vi "FluidtekPrensaCONidentLEDI_v15.vi"() -> ()   [LabVIEW 2026]
uses:
  <vilib>/DAQmx/read.llb/DAQmx Read (Digital 1D Bool NChan 1Samp 1Line).vi
  <vilib>/DAQmx/write.llb/DAQmx Write (Digital 1D Bool NChan 1Samp 1Line).vi
  <vilib>/DAQmx/read.llb/DAQmx Read (Analog 1D Wfm NChan NSamp).vi
  <vilib>/Analysis/baseanly.llb/Mean (DBL).vi
  <vilib>/DAQmx/write.llb/DAQmx Write (Analog DBL 1Chan 1Samp).vi
  <extravilib>/ChannelInstances/Tag-bool/Read With Abort.vi
  <extravilib>/ChannelInstances/Tag-c(dbl,dbl,dbl,dbl,dbl,dbl)/Read With Abort.vi
  <extravilib>/ChannelInstances/Tag-c(dbl,dbl,dbl,dbl,dbl,dbl,dbl,bool,u16)/Write With Abort.vi
  <extravilib>/ChannelInstances/Tag-bool/Write With Abort.vi
  <extravilib>/ChannelInstances/Tag-c(dbl,dbl,dbl,dbl,dbl,dbl,dbl,bool,u16)/Read With Abort.vi
  <extravilib>/ChannelInstances/Tag-c(dbl,dbl,dbl,dbl,dbl,dbl)/Write With Abort.vi
  GlobalesPrensa.vi
  <vilib>/Utility/file.llb/Write Delimited Spreadsheet (DBL).vi
  <vilib>/DAQmx/create/channels.llb/DAQmx Create Channel (AO-Voltage-Basic).vi
  <vilib>/DAQmx/create/channels.llb/DAQmx Create Channel (AI-Voltage-Basic).vi
  <vilib>/DAQmx/configure/timing.llb/DAQmx Timing (Sample Clock).vi
  <vilib>/DAQmx/create/channels.llb/DAQmx Create Channel (DO-Digital Output).vi
  <vilib>/DAQmx/create/channels.llb/DAQmx Create Channel (DI-Digital Input).vi
  <extravilib>/ChannelInstances/Tag-bool/Instantiate.vi
  <extravilib>/ChannelInstances/Tag-bool/Endpoint.vi
  <vilib>/DAQmx/miscellaneous.llb/DAQmx Fill In Error Info.vi
  <extravilib>/ChannelInstances/Tag-c(dbl,dbl,dbl,dbl,dbl,dbl,dbl,bool,u16)/Instantiate.vi
  <extravilib>/ChannelInstances/Tag-c(dbl,dbl,dbl,dbl,dbl,dbl)/Instantiate.vi
  <extravilib>/ChannelInstances/Tag-bool/EndpointRead.vi
  <extravilib>/ChannelInstances/Tag-c(dbl,dbl,dbl,dbl,dbl,dbl)/EndpointRead.vi
  <extravilib>/ChannelInstances/Tag-c(dbl,dbl,dbl,dbl,dbl,dbl,dbl,bool,u16)/Endpoint.vi
  <extravilib>/ChannelInstances/Tag-c(dbl,dbl,dbl,dbl,dbl,dbl,dbl,bool,u16)/EndpointRead.vi
  <extravilib>/ChannelInstances/Tag-c(dbl,dbl,dbl,dbl,dbl,dbl)/Endpoint.vi
  <vilib>/Analysis/NI_AALBase.lvlib
  <extravilib>/ChannelInstances/Tag-bool.lvlib
  <extravilib>/ChannelInstances/Tag-c(dbl,dbl,dbl,dbl,dbl,dbl).lvlib
  <vilib>/ptbypt/NI_PtbyPt.lvlib
  <extravilib>/ChannelInstances/Tag-c(dbl,dbl,dbl,dbl,dbl,dbl,dbl,bool,u16).lvlib
panel:
  out "Archivo":path
  out "Lg log":dbl[](array[numeric])
  in  "PARO DE EMERGENCIA":bool
  out "time/iteration (ms)":u32=210
  in  "Tab Control 3":enum32{"ENSAYO", "REGISTRO"}(tab)
  in  "Tipo ensayos":u16(ring)=1 items=["Flexotraccion en losas", "Tenacidad Vigas"]
  in  "Rampa (mm/min)":dbl=0.1 min=0.0 max=25.0 format="%.3f"
  in  "Rampa (kN/min)":dbl=0.1 min=0.0 max=20.0 format="%.2f"
  in  "Limite fuerza (kN)":dbl=3.0 min=0.0 max=150.0 format="%.2f"
  in  "Limite posicion (mm)":dbl=145.0 min=0.0 max=150.0 format="%.2f"
  in  "Tiempo carga (s)":dbl=3.0 min=0.0 max=300.0 format="%.2g"
  out "Tiempo (s)":dbl format="%.2f"
  in  "Iniciar ensayo":bool
  out "Velocidad norma (mm/min)  2":string="0.05 - 0.1"
  in  "Tenacidad en vigas":u16(ring) items=["ASTM 1609 con100x100x350", "ASTM 1609 con150x150x500", "EFNARC 1996", "VIGAS 14651", "ENS. BARCELONA"]
  in  "Aplicar velocidad de norma":bool
  out "Estado del ensayo":dbl(ring) items=["REPOSO", "CARGA (rampa)", "MANTENIENDO CARGA", "DESCARGA", "RETORNO / FIN", "FALLA - ENSAYO DETENIDO", ""]
  in  "Flexotracción en losas":u16(ring)=3 items=["EFNARC 1996", "EFNARC 1999", "EFNARC 14488-5", "ASTM 1550"]
  out "Velocidad norma (mm/min)":dbl=4.0
  in  "IPAddress QuantumX":string="172.31.236.115"
  out "LicenseIsValid":bool
  in  "Registrar":bool
  in  "ID manual (0=auto)":i32
  in  "Tipo":string
  in  "INFLE":dbl
  in  "Detener registro":bool
  in  "Tab Control 2":T1(tab)
  out "Presión B (bar)":dbl=31.47939829954219 format="%.2f"
  out "Presión A (bar)":dbl=47.7049180327869 format="%.2f"
  out "Vertical Progress Bar":dbl(slide)=3.0
  in  "Tab Control":enum32{"Desplazamiento", "Fuerza"}(tab)
  in  "PID fuerza":T2={"proportional gain (Kc)"=1.0, "integral time (Ti, min)"=0.03, "derivative time (Td, min)"=0.0} {"derivative time (Td, min)" format="%.3f"; "integral time (Ti, min)" format="%.3f"; "proportional gain (Kc)" format="%.3f"}
  out "control signals":dynamicdata(graph)=[{"t0"=timestamp(3594752785.1434503 s since 1904-01-01), "dt"=1.0, "Y"=[3.0]}, {"t0"=timestamp(3594752785.1434503 s since 1904-01-01), "dt"=1.0, "Y"=[3.0680651042487943]}]
  in  "Posicion deseada (mm)":dbl(slide)=3.0 min=2.0 max=150.0 scale format="%#_2f"
  in  "Fuerza deseada (kN)":dbl=0.5 min=0.0 max=150.0 format="%.2f"
  out "Fuerza actual (KN)":dbl format="%.2f"
  out "Posicion actual (mm)":dbl format="%.2f"
  in  "Tipo control":u16(ring) items=["Desplazamiento", "Fuerza"]
  out "fuerza desplazamiento":cluster{dbl[], dbl[]}(graph)
  out "Rigidez estimada (kN/mm)":dbl
  out "Carga maxima (kN)":dbl
  out "Progreso mantenimiento":dbl(slide) scale=0.0..100.0
  out "Tiempo restante carga (s)":dbl
  out "Falla":bool
  out "Causa de la falla":dbl(ring) items=["Sin falla", "CAIDA DE CARGA (rotura)", "SOBRECARGA", "LIMITE DE POSICION", "PARO DE EMERGENCIA", "LIMITE DEL SISTEMA (160 kN)", "SIN LECTURA DE FUERZA (QuantumX)", "LIMITE POR PRESIONES (160 kN)"]
  out "Proteccion de fuerza activa":bool
  in  "Vel. aproximacion (mm/min)":dbl=50.0 min=0.1 max=50.0
  in  "Fmax fuera de ensayo (kN)":dbl=1.0 min=0.2 max=50.0
  out "UPH energizada":bool=TRUE
  out "Nivel tanque":bool
  out "Estado de  filtro":bool=TRUE
  out "Sobrecorriente":bool
  in  "Stop":bool
  out "Estado de motor":bool
  in  "Apagar":bool
  in  "Encender":bool
  in  "Sin proteccion de carga":bool
  in  "Confirmar parametros":bool=TRUE
  out "Consigna posicion interna (mm)":dbl
  out "Parametros avanzados":dbl(ring) items=["POR DEFECTO (bloqueados)", "PERSONALIZADOS (activos)"]
  in  "Codigo acceso":dbl
  in  "Sobrecarga falla (x limite)":dbl=1.2
  in  "Caida para falla (0-1)":dbl=0.3
  in  "Rigidez inicial (kN/mm)":dbl=1.0
  in  "Kf lazo fuerza (1/s)":dbl=0.5
  in  "Kx lazo posicion (V/mm)":dbl=30.0
  in  "Ti lazo posicion (s)":dbl=1.5
  # "PB"
  # "PA"
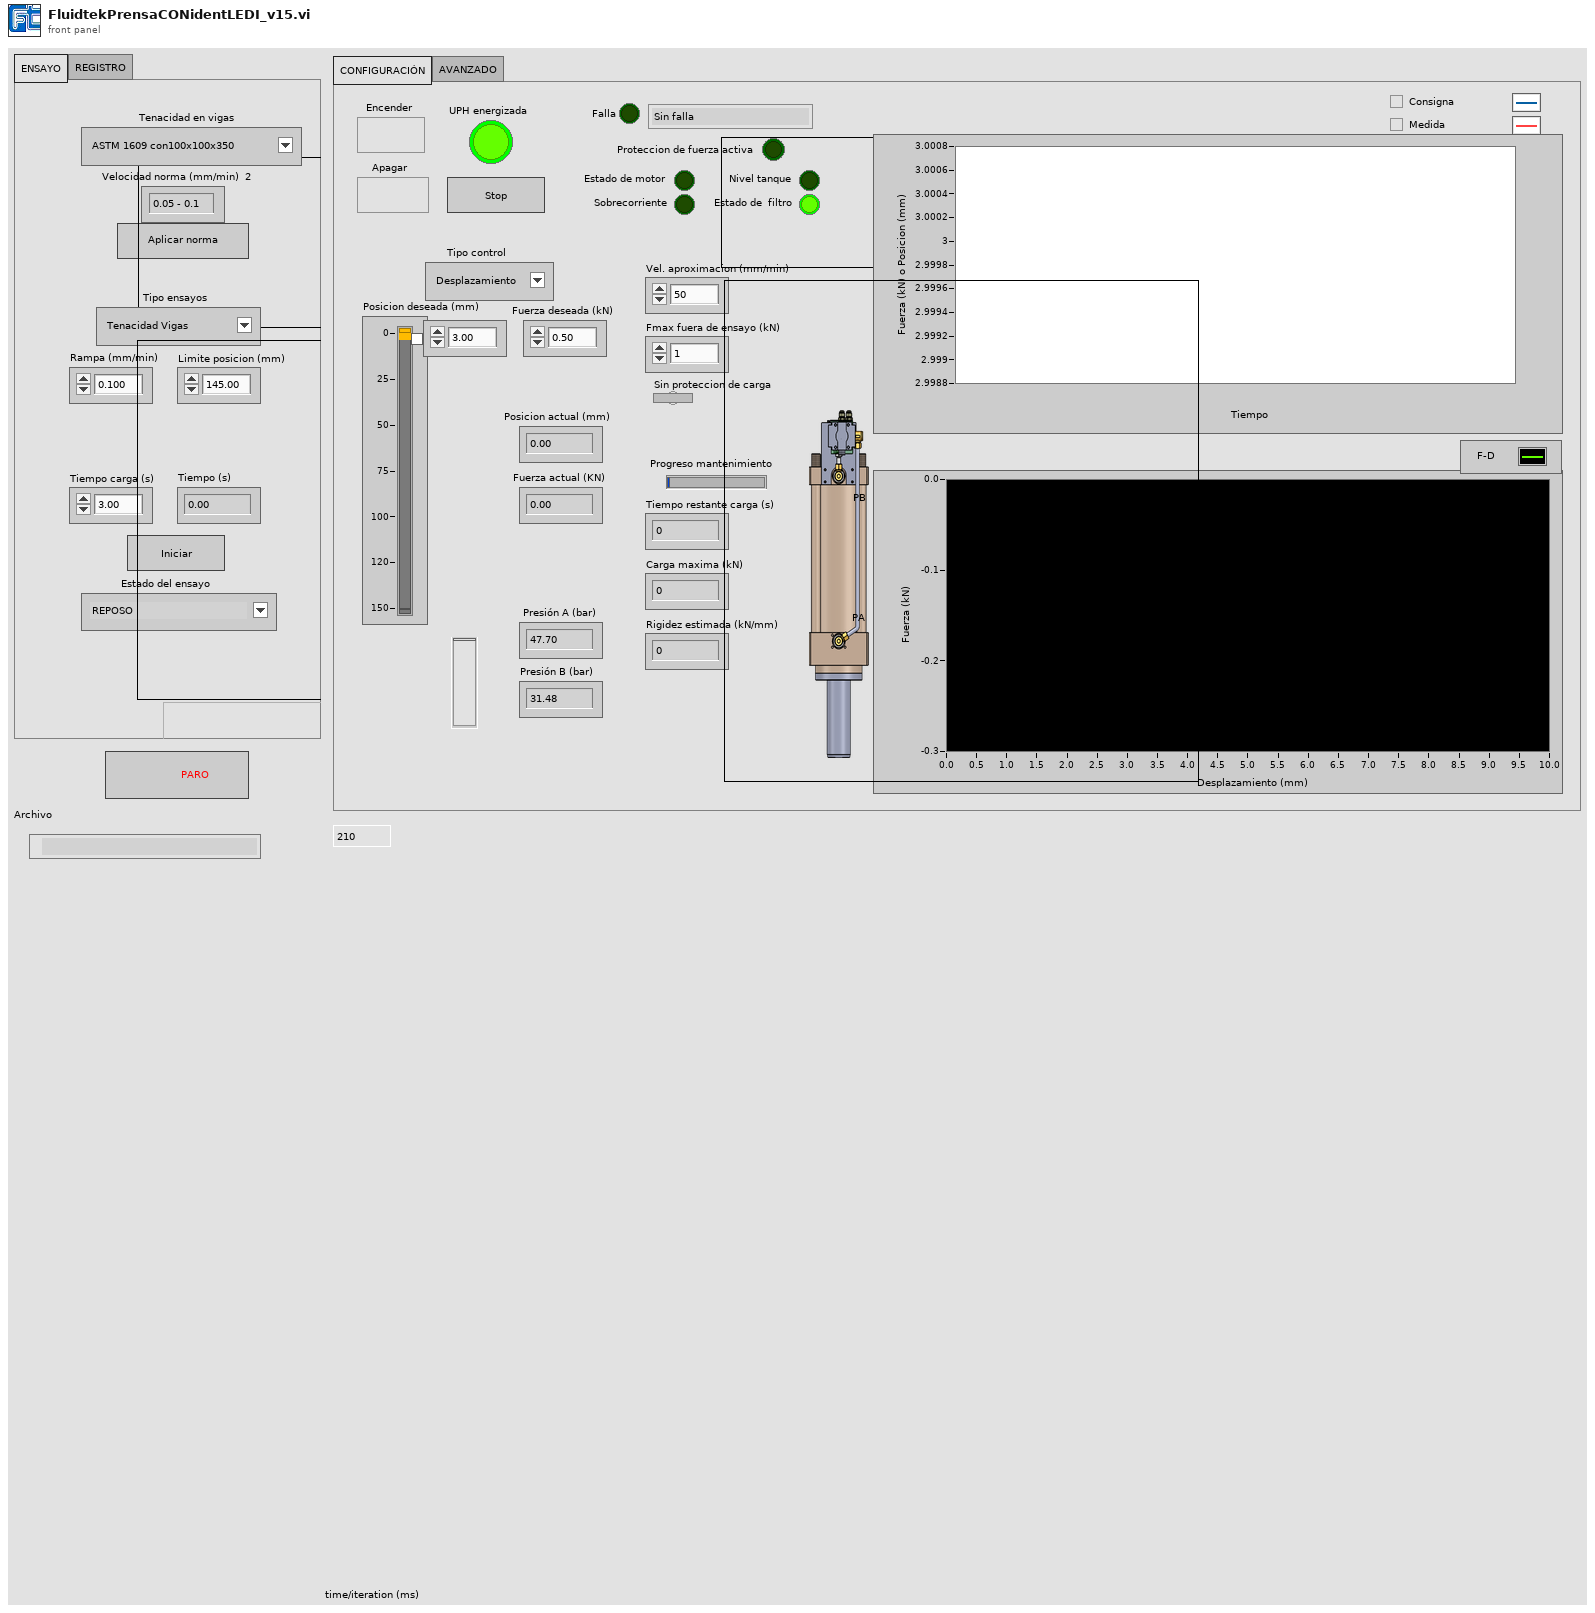
[diagram p1: front panel]
types:
  T1 = enum32{"CONFIGURACIÓN", "AVANZADO", "identificación (no modificar)"}
  T2 = cluster{"proportional gain (Kc)":dbl, "integral time (Ti, min)":dbl, "derivative time (Td, min)":dbl}
  T3 = typedef "Tag-bool.lvlib/))Channel.ctl" = refnum<queue>
  T4 = cluster{"Devices":refnum<k24>[], "Signals":refnum<k24>[]}
  T5 = cluster{"Rampa (mm/min)":dbl, "Rampa (kN/min)":dbl, "Limite posicion (mm)":dbl, "Limite fuerza (kN)":dbl, "Posicion deseada (mm)":dbl, "Fuerza deseada (kN)":dbl, "Tiempo carga (s)":dbl, "Iniciar ensayo":bool, "Tipo control":u16}
  T6 = cluster{"Numeric":dbl, "mean":dbl, "mean":dbl, "mean":dbl, "mean":dbl, "sp":dbl}
  T7 = typedef "Tag-c(dbl,dbl,dbl,dbl,dbl,dbl).lvlib/))Channel.ctl" = refnum<queue>
  T8 = enum8{"Enabled", "Disabled", "Disabled and Grayed Out"}
  T9 = cluster{"Numeric":dbl, dbl, dbl, dbl, dbl, "Limite fuerza (kN)":dbl}
  T10 = typedef "Tag-c(dbl,dbl,dbl,dbl,dbl,dbl,dbl,bool,u16).lvlib/))Channel.ctl" = refnum<queue>
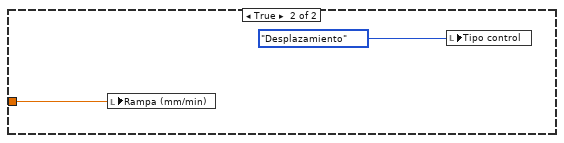
[diagram p5: hidden frame]
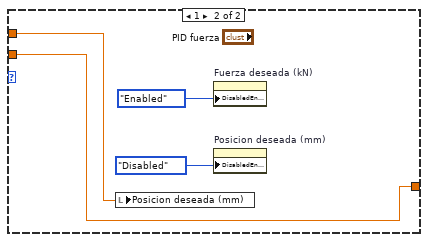
[diagram p6: hidden frame]
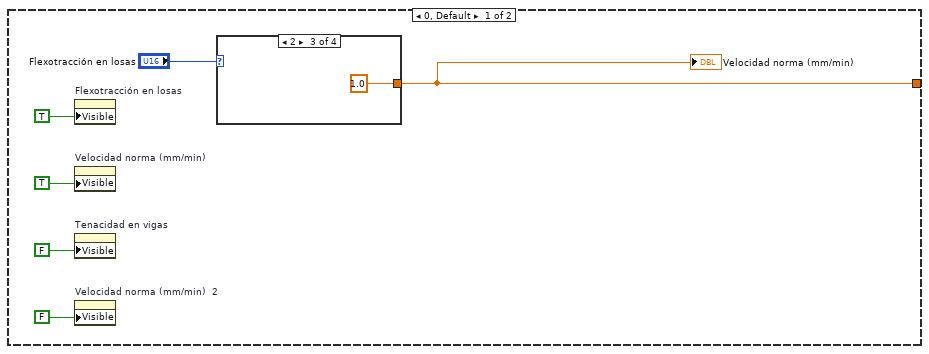
[diagram p7: hidden frame]
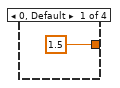
[diagram p8: hidden frame]
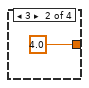
[diagram p9: hidden frame]
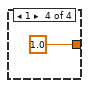
[diagram p10: hidden frame]
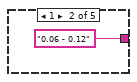
[diagram p11: hidden frame]
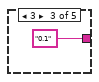
[diagram p12: hidden frame]
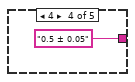
[diagram p13: hidden frame]
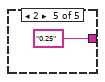
[diagram p14: hidden frame]
diagram:
  w76 = 0 items=["one channel for each line", "one channel for all lines"] ("line grouping")
  w83 = 0 items=["one channel for each line", "one channel for all lines"] ("line grouping")
  w95 = 10348 items=["Volts"=10348, "From Custom Scale"=10065] ("units")
  w98 = -1 items=["Default"=-1, "RSE"=10083, "NRSE"=10078, "Differential"=10106, "Pseudodifferential"=12529] ("input terminal configuration")
  w106 = 10348 items=["Volts"=10348, "From Custom Scale"=10065] ("units")
  w104 = 10106 items=["Default"=-1, "RSE"=10083, "NRSE"=10078, "Differential"=10106, "Pseudodifferential"=12529] ("input terminal configuration")
  w100 = 10123 items=["Finite Samples"=10178, "Continuous Samples"=10123, "Hardware Timed Single Point"=12522] ("sample mode")
  # "Convert device reference to array of device references\n(since ConnectDevice.vi expects an array of devices)..."
  # "Disconnect devices"
  # "Set samplerate and filter frequency for all selected signals."
  # "Initialize HBM Common API for LabVIEW"
  # "End API usage"
  # "Stop DAQ"
  # "Run data acquisition for 10 sec. DAQ-loop: Update signals and do anything with the  measurement values.\n(Here: show first signal in diagram)"
  # "Start DAQ"
  # "Prepare DAQ"
  # "v14: senales [0,1,2,3] -> lazo lee 1,2,3 = W100 (conector 2), Tempsonic (conector 3), Celda via Krenel (conector 4). Filtro 20 Hz, 50 Hz"
  # "Get all signals of the devices"
  # "Connect devices"
  # "Use certain QuantumX device"
  # "Assign the signals...."
  # "Vel. aprox. (mm/min)"
  # "LAZO E/S DIGITAL: encendido/apagado de la unidad hidraulica (contactores), lectura de alarmas (motor, sobrecorriente, nivel, filtro)."
  # "LAZO HMI: lee el panel, habilita/oculta controles segun modo y estado, envia consignas al lazo de control por canal (Tag)."
  # "LAZO DE CONTROL: lectura DAQ (fuerza, desplazamiento, presiones) -> Formula Node 'CONTROLADOR' (maquina de estados + cascada fuerza/posicion + fallas) -> salida servovalvula (AO). Parametros avanzados protegidos con codigo."
  n1 = while {
    tunnel: [w111] -> w3
    tunnel: [w111] -> w2
    tunnel: [w111] -> w1
    i -> [w116]
    stop <- w114 continue-if-true
    n2 = call <vilib>:"DAQmx Reserve Network Device.vi"("device in"=tag "cDAQ9184-1ADC24C", "override reservation?"=TRUE, "error in"=errorcluster {"status"=FALSE, "code"=0, "source"=""}) -> ("error out"=w111:errorcluster)  [unwired: 11 in, 1 out]
    n3 = Unbundle By Name(w111) -> ("status"=w113:bool)
    n4 = Less?(x=w116, y=30) -> (x < y?=w115:bool)
    n5 = And(x=w113, y=w115) -> (x .and. y?=w114:bool)
    n6 = Wait (ms)(milliseconds to wait=u32 2000) -> ()  [unwired: 1 out]
  }
  n7 = call-poly <vilib>:"DAQmx Create Virtual Channel.vi"("lines"=tag "PrensaLEDI_DO/port0/line0:7", "line grouping"=w76, "error in"=w2) -> ("task out"=w77:refnum<k21>, "error out"=w78:errorcluster)  [unwired: 11 in]
  n8 = call-poly <vilib>:"DAQmx Create Virtual Channel.vi"("lines"=tag "PrensaLEDI_DI/port0/line0:7", "line grouping"=w83, "error in"=w3) -> ("task out"=w80:refnum<k21>, "error out"=w81:errorcluster)  [unwired: 11 in]
  n9 = call <vilib>:"DAQmx Start Task.vi"("task/channels in"=w77, "error in"=w78) -> ("task out"=w71:refnum<k21>, "error out"=w70:errorcluster)  [unwired: 12 in]
  n10 = call <vilib>:"DAQmx Start Task.vi"("task/channels in"=w80, "error in"=w81) -> ("task out"=w73:refnum<k21>, "error out"=w72:errorcluster)  [unwired: 12 in]
  n11 = while {
    tunnel: w73 -> [w132]
    tunnel: w72 -> [w131]
    tunnel: [w130] -> w56
    tunnel: [w129] -> w54
    tunnel: w71 -> [w128]
    tunnel: [w127] -> w60
    tunnel: w70 -> [w126]
    tunnel: [w125] -> w58
    tunnel: [w124] -> w6
    stop <- "Stop" stop-if-true
    # "6"
    # "APAGADO Y ENCENDIDO TIPO PULSO"
    # "transmisor de presion"
    # "salida contactor2"
    # "salida al contactor"
    # "pulsador\nemergencia"
    # "GM2"
    n12 = call-poly <vilib>:"DAQmx Read.vi"("task/channels in"=w132, "error in"=w131) -> ("task out"=w130:refnum<k21>, "data"=w147:bool[], "error out"=w129:errorcluster)  [unwired: 11 in]
    n13 = Index Array(array=w147, index=7) -> ()  [unwired: 1 out]
    n14 = global write "GlobalesPrensa.vi" "Salir"("Stop") -> ()
    n15 = Index Array(array=w147, index=5) -> (element=w156:bool)
    "Sobrecorriente" <- w156
    n16 = Index Array(array=w147, index=0) -> (element=w146:bool)
    n17 = Index Array(array=w147, index=2) -> (element=w148:bool)
    n18 = Not(x="Stop") -> (.not. x?=w145:bool)
    n19 = Not(x=w148) -> (.not. x?=→"Estado de  filtro":bool)
    n20 = Not(x=w156) -> (.not. x?=→"UPH energizada":bool)
    n21 = And(x=w146, y=w145) -> (x .and. y?=w152:bool)
    n22 = Index Array(array=w147, index=1) -> (element=→"Nivel tanque":bool)
    n23 = local read "PARO DE EMERGENCIA"() -> (w121:bool)
    n24 = Not(x=w152) -> (.not. x?=w153:bool)
    n25 = Not(x=w152) -> (.not. x?=w154:bool)
    n26 = Or(x="Apagar", y=w153) -> (x .or. y?=w122:bool)
    n27 = Or(x=w122, y=w121) -> (x .or. y?=w123:bool)
    n28 = while {
      shift-right: [w160] -> w157
      shift-left: _ -> [w162]
      tunnel: "Encender" -> [w161]
      tunnel: w123 -> [w159]
      stop <- FALSE continue-if-true
      n29 = Exclusive Or(1:w159, 2:w161) -> (0:w163:bool)
      n30 = Select(t=w161, s=w163, f=w162) -> (s? t:f=w160:bool)
    }
    "Estado de motor" <- w157
    n31 = Wait (ms)(milliseconds to wait=u32 500) -> ()  [unwired: 1 out]
    n32 = Replace Array Subset(array=bool[] [FALSE, FALSE, FALSE, FALSE, FALSE, FALSE, FALSE, FALSE], new element #1=w157, index #1=0 ("index"), new element #2=w154, index #2=2 ("index"), new element #3=TRUE ("new element/subarray"), index #3=5 ("index")) -> (w155:bool[])
    n33 = call-poly <vilib>:"DAQmx Write.vi"("task/channels in"=w128, "data"=w155, "error in"=w126) -> ("task out"=w127:refnum<k21>, "error out"=w125:errorcluster)  [unwired: 10 in, 1 out]
    n34 = call <extravilib>:"Write.vi"("element"="Stop") -> ("channel"=w124:T3)  [unwired: 1 out]
  }
  n35 = call-poly <vilib>:"DAQmx Create Virtual Channel.vi"("maximum value"=10.0, "minimum value"=0.0, "input terminal configuration"=w104, "physical channels"=tag "PrensaLEDI_AI/ai0:3", "units"=w106, "error in"=w1) -> ("task out"=w107:refnum<k21>, "error out"=w108:errorcluster)  [unwired: 8 in]
  n36 = call-poly <vilib>:"DAQmx Create Virtual Channel.vi"("maximum value"=10.0, "minimum value"=-10.0, "output terminal configuration"=w98, "physical channels"=tag "PrensaLEDI_AO/ao0", "units"=w95, "error in"=w1) -> ("task out"=w99:refnum<k21>, "error out"=w97:errorcluster)  [unwired: 8 in]
  n37 = call-poly <vilib>:"DAQmx Timing.vi"("task/channels in"=w107, "sample mode"=w100, "samples per channel"=500000, "rate"=200000.0, "error in"=w108) -> ("task out"=w68:refnum<k21>, "error out"=w67:errorcluster)  [unwired: 9 in]
  n38 = call <vilib>:"DAQmx Start Task.vi"("task/channels in"=w68, "error in"=w67) -> ("task out"=w66:refnum<k21>, "error out"=w65:errorcluster)  [unwired: 12 in]
  n39 = call <vilib>:"DAQmx Start Task.vi"("task/channels in"=w99, "error in"=w97) -> ("task out"=w88:refnum<k21>, "error out"=w87:errorcluster)  [unwired: 12 in]
  n40 = feedback-in #1(w6) -> ()
  n41 = feedback #1() -> ()  [unwired: 2 in]
  n42 = call <vilib>:"DAQmx Stop Task.vi"("task/channels in"=w60, "error in"=w58) -> ("task out"=w59:refnum<k21>, "error out"=w57:errorcluster)  [unwired: 12 in]
  n43 = call <vilib>:"DAQmx Stop Task.vi"("task/channels in"=w56, "error in"=w54) -> ("task out"=w55:refnum<k21>, "error out"=w53:errorcluster)  [unwired: 12 in]
  n44 = call <vilib>:"DAQmx Clear Task.vi"("task in"=w59, "error in"=w57) -> ("error out"=w75:errorcluster)  [unwired: 13 in]
  n45 = call <vilib>:"DAQmx Clear Task.vi"("task in"=w55, "error in"=w53) -> ("error out"=w74:errorcluster)  [unwired: 13 in]
  n46 = call <vilib>:"Simple Error Handler.vi"("error in (no error)"=w75) -> ()  [unwired: 4 in, 5 out]
  n47 = call <vilib>:"Simple Error Handler.vi"("error in (no error)"=w74) -> ()  [unwired: 4 in, 5 out]
  n48 = call <userlib>:"Init.vi"() -> ("LicenseIsValid"=→"LicenseIsValid":bool, "Error out"=w13:errorcluster)  [unwired: 8 in, 1 out]
  n49 = call <userlib>:"QuantumX_Device.vi"("Error in"=w13, "IPAddress"="IPAddress QuantumX") -> ("Error out"=w14:errorcluster, "Device"=w11:refnum<k24>)  [unwired: 6 in]
  n50 = Build Array(w11) -> (w10:refnum<k24>[])
  n51 = call <userlib>:"ConnectDevice.vi"("Error in"=w14, "Devices"=w10) -> ("Error out"=w36:errorcluster, "Devices"=w35:refnum<k24>[])  [unwired: 7 in, 1 out]
  n52 = call <userlib>:"GetSignals.vi"("Error in"=w36, "Devices"=w35) -> ("Error out"=w30:errorcluster, "DevicesAndSignals"=w31:T4)  [unwired: 8 in]
  n53 = Unbundle By Name(w31) -> ("Devices"=w24:refnum<k24>[], "Signals"=w28:refnum<k24>[])
  n54 = Index Array(array=w28, index #1=0 ("Index"), index #2=1 ("Index"), index #3=2 ("Index"), index #4=3 ("Index")) -> (element #1=w27:refnum<k24>, element #2=w26:refnum<k24>, element #3=w19:refnum<k24>, element #4=w18:refnum<k24>)
  n55 = Build Array(w27, w26, w19, w18) -> (w25:refnum<k24>[])
  n56 = Bundle(cluster=w31, "Devices"=w24, "Signals"=w25) -> (w32:T4)
  n57 = Unbundle By Name(w32) -> ("Signals"=w48:refnum<k24>[])
  n58 = case shown="No Error" w30 {
    tunnel: w30 -> [w169 w175]
    tunnel: w48 -> [w168 _]
    tunnel: [w167 w175] -> w47
    frame No Error {
      # "Filter frequency:"
      # "Samplerate:"
      n59 = for {
        tunnel: w169 -> [w174]
        tunnel: 50.0 ("SampleRate") -> [w173]
        tunnel: 20.0 ("FilterFrequency") -> [w172]
        tunnel: w168 -> [w171] mode=indexing
        tunnel: [w170] -> w167
        stop <- w170 stop-if-true
        n60 = call <userlib>:"ConfigSignal.vi"("Error in"=w174, "SampleRate"=w173, "FilterFrequency"=w172, "Signal"=w171) -> ("Error out"=w170:errorcluster)  [unwired: 7 in]
      }
    }
    frame Error {
    }
  }
  n61 = call <userlib>:"AssignSignals.vi"("Error in"=w47, "DevicesAndSignals"=w32) -> ("Error out"=w45:errorcluster, "DevicesAndSignals"=w46:T4)  [unwired: 8 in]
  n62 = call <userlib>:"PrepareDAQ.vi"("Error in"=w45, "DevicesAndSignals"=w46) -> ("Error out"=w42:errorcluster, "DaqMeasurement"=w43:refnum<k24>, "DevicesAndSignals"=w44:T4)  [unwired: 7 in]
  n63 = call <userlib>:"StartDaq.vi"("DevicesAndSignals"=w44, "DaqMeasurement"=w43, "AcquisitionMode"=2, "Error in"=w42) -> ("DevicesAndSignals"=w39:T4, "DaqMeasurement"=w40:refnum<k24>, "Error out"=w41:errorcluster)  [unwired: 7 in, 2 out]
  n64 = while {
    tunnel: w40 -> [w236]
    tunnel: w39 -> [w235]
    tunnel: [w231] -> w38
    tunnel: [w230] -> w37
    tunnel: w41 -> [w237]
    tunnel: [w229] -> w5
    shift-right: [w197] -> _
    shift-left: 0 -> [w222]
    shift-right: [w188] -> _
    shift-left: FALSE ("Registrar") -> [w193]
    shift-right: [w192] -> _
    shift-left: _ -> [w194]
    stop <- w183 stop-if-true
    n65 = global read "GlobalesPrensa.vi" "Salir"() -> (w182:bool)
    n66 = Get Date/Time In Seconds() -> (seconds since 1Jan1904=w205:timestamp)
    n67 = Format Into String(format string="D:\\\\%<%Y>T\\\\%03d-%<%Y>T", w205, "INFLE", w205) -> (resulting string=w207:string)  [unwired: 2 in, 1 out]
    n68 = Or(x=w182, y="Detener registro") -> (x .or. y?=w183:bool)
    n69 = String To Path(string=w207) -> (path=w210:path)
    n70 = Create Folder(path (use dialog)=w210) -> (error out=w208:errorcluster)  [unwired: 2 in, 2 out]
    n71 = Format Into String(format string="%s P*", "Tipo") -> (resulting string=w211:string)  [unwired: 2 in, 1 out]
    n72 = call <vilib>:"Clear Errors.vi"("error in (no error)"=w208) -> ("error out"=w209:errorcluster)  [unwired: 5 in, 1 out]
    n73 = List Folder(path=w210, pattern=w211, error in=w209) -> (path out=w220:path, filenames=w212:string[])  [unwired: 1 in, 2 out]
    n74 = Not(x=w193) -> (.not. x?=w199:bool)
    n75 = for {
      tunnel: w212 -> [w264] mode=indexing
      tunnel: [w262] -> w213 mode=indexing
      n76 = Scan From String(format string="%s P%d", input string=w264) -> (error out=w261:errorcluster, output 2=w262:i32)  [unwired: 5 in, 2 out]
      n77 = call <vilib>:"Clear Errors.vi"("error in (no error)"=w261) -> ()  [unwired: 5 in, 2 out]
    }
    n78 = Array Max & Min(array=w213) -> (max value=w214:i32)  [unwired: 3 out]
    n79 = Greater Than 0?(x="ID manual (0=auto)") -> (x > 0?=w216:bool)
    n80 = Increment(x=w214) -> (x+1=w215:i32)
    n81 = Select(t="ID manual (0=auto)", s=w216, f=w215) -> (s? t:f=w218:i32)
    n82 = global read "GlobalesPrensa.vi" "Ensayando"() -> (w189:bool)
    n83 = global read "GlobalesPrensa.vi" "InfoEnsayo"() -> (w186:string)
    n84 = Format Into String(format string="%s P%d.csv", "Tipo", w218) -> (resulting string=w219:string)  [unwired: 2 in, 1 out]
    n85 = Or(x="Registrar", y=w189) -> (x .or. y?=w188:bool)
    n86 = Build Path(base path=w220, name or relative path=w219) -> (appended path=w195:path)
    n87 = Get Date/Time In Seconds() -> (seconds since 1Jan1904=w187:timestamp)
    n88 = And(x=w188, y=w199) -> (x .and. y?=w200:bool)
    n89 = Select(t=w194, s=w193, f=w195) -> (s? t:f=w192:path)
    "Archivo" <- w192
    n90 = Format Into String(format string="Fecha\t%<%Y-%m-%d %H:%M:%S>T\nNorma\t%s\nFrecuencia (Hz)\t50\nRunning Time\tDeflection\tDisplacement\tLoad\ns\tmm\tmm\tkN\n", w187, w186) -> (resulting string=w185:string)  [unwired: 2 in, 1 out]
    n91 = case shown="True" w200 {
      tunnel: [_ w259] -> w201
      tunnel: w192 -> [_ w257]
      tunnel: w185 -> [_ w258]
      frame False {
      }
      frame True {
        (unwired) "" ("text")
        (unwired) errorcluster {"status"=FALSE, "code"=0, "source"=""} ("error in")
        (unwired) "" ("prompt (Choose or enter file path)")
        # "t (s)\\testado\\tconsigna\\tF (kN)\\tx (mm)\\txsp (mm)\\tu (V)\\tkh (kN/mm)\\tdt (s)\\tfalla\\tcausa\\tprot\\n"
        n92 = Path To String(path=w257) -> (string=w256:string)
        n93 = Search and Replace String(replace all?=FALSE ("replace all? (F)"), case sensitive?=FALSE ("ignore case? (F)"), input string=w256, search string=".csv", replace string="_control.csv" ("replace string (\"\")"), offset=0 ("offset (0)"), error in=errorcluster {"status"=FALSE, "code"=0, "source"=""} ("error in (no error)")) -> (result string=w249:string)  [unwired: 1 in, 3 out]
        n94 = String To Path(string=w249) -> (path=w248:path)
        n95 = Write to Text File(file (use dialog)=w248, text="t (s)\testado\tconsigna\tF (kN)\tx (mm)\txsp (mm)\tu (V)\tkh (kN/mm)\tdt (s)\tfalla\tcausa\tprot\tpA (bar)\tpB (bar)\tFp (kN)\n") -> (error out=w246:errorcluster)  [unwired: 2 in, 2 out]
        n96 = flat-sequence {
          tunnel: w248 -> [w260]
          tunnel: w246 -> [_]
          frame #0 {
            n97 = global write "GlobalesPrensa.vi" "ArchivoControl"(w260) -> ()
          }
        }
        n98 = Write to Text File(file (use dialog)=w257, text=w258) -> (error out=w259:errorcluster)  [unwired: 2 in, 2 out]
      }
    }
    n99 = call <userlib>:"UpdateMeasurementValues.vi"("Error in"=w237, "DaqMeasurement"=w236, "DevicesAndSignals"=w235) -> ("Error out"=w232:errorcluster, "DaqMeasurement"=w233:refnum<k24>, "DevicesAndSignals"=w234:T4)  [unwired: 6 in]
    n100 = for {
      N: 3 -> [_]
      shift-right: [w276] -> w230
      shift-left: w234 -> [w280]
      shift-right: [w277] -> w231
      shift-left: w233 -> [w279]
      shift-right: [w275] -> w229
      shift-left: w232 -> [w278]
      tunnel: [w270] -> w181 mode=indexing
      i -> [w273]
      n101 = Add(x=w273, y=1.0) -> (x+y=w272:dbl)
      n102 = call <userlib>:"GetMeasurementValues.vi"("Error in"=w278, "Index"=w272, "DaqMeasurement"=w279, "DevicesAndSignals"=w280) -> ("Error out"=w275:errorcluster, "Waveform"=w271:waveform(dbl), "DaqMeasurement"=w277:refnum<k24>, "DevicesAndSignals"=w276:T4)  [unwired: 2 in, 2 out]
      n103 = Unbundle By Name(w271) -> ("Y"=w270:dbl[])
    }
    n104 = feedback #2() -> (w179:dbl)  [unwired: 1 in]
    n105 = Tick Count (ms)() -> (millisecond timer value=w180:u32)
    n106 = Array Size(array=w181) -> (size(s)=w225:i32[])
    n107 = Index Array(array=w225, index=1) -> (element=w223:i32)
    n108 = for {
      N: w223 -> [_]
      tunnel: [w267] -> w221 mode=indexing
      tunnel: w222 -> [w265]
      i -> [w269]
      n109 = Add(x=w269, y=w265) -> (x+y=w268:i32)
      n110 = Multiply(x=w268, y=0.02) -> (x*y=w267:dbl)
    }
    n111 = Add(x=w222, y=w223) -> (x+y=w198:i32)
    n112 = feedback #3() -> (w178:dbl)  [unwired: 1 in]
    n113 = formula code="int32 n,m; m=sizeOfDim(D,0); n=sizeOfDim(D,1);\nif (m>2 && n>0) { Fq=D[2][n-1]; tq=tk; } else { Fq=Fo; tq=to; }"("D"=w181, "tk"=w180, "Fo"=w179, "to"=w178) -> ("Fq"=w177:dbl, "tq"=w176:dbl)
    n114 = feedback-in #2(w177) -> ()
    n115 = global write "GlobalesPrensa.vi" "F_QX"(w177) -> ()
    n116 = global write "GlobalesPrensa.vi" "tQX"(w176) -> ()
    n117 = feedback-in #3(w176) -> ()
    n118 = Select(t=w198, s=w188, f=0) -> (s? t:f=w197:i32)
    n119 = case shown="True" w188 {
      tunnel: w181 -> [_ w245]
      tunnel: w221 -> [_ w244]
      tunnel: w201 -> [_ w239]
      tunnel: w192 -> [_ w238]
      frame False {
      }
      frame True {
        n120 = Insert Into Array(array=w245, index (row)=0, new element=w244) -> (w242:dbl[][])  [unwired: 1 in]
        n121 = call-poly <vilib>:"Write Delimited Spreadsheet.vi"("file path (dialog if empty)"=w238, "2D data"=w242, "append to file? (new file:F)"=TRUE, "error in (no error)"=w239, "transpose? (no:F)"=TRUE) -> ()  [unwired: 9 in, 2 out]
      }
    }
    n122 = Wait Until Next ms Multiple(millisecond multiple=u32 20 ("Vielfache von ms")) -> ()  [unwired: 1 out]
  }
  n123 = call <vilib>:"Clear Errors.vi"("error in (no error)"=w5) -> ("error out"=w4:errorcluster)  [unwired: 5 in, 1 out]
  n124 = call <userlib>:"StopDaq.vi"("Error in"=w4, "DaqMeasurement"=w38, "DevicesAndSignals"=w37) -> ("Error out"=w17:errorcluster, "DevicesAndSignals"=w16:T4)  [unwired: 7 in]
  n125 = call <userlib>:"DisconnectDevice.vi"("Error in"=w17, "DevicesAndSignals"=w16) -> ("Error out"=w15:errorcluster)  [unwired: 9 in]
  n126 = call <vilib>:"Simple Error Handler.vi"("error in (no error)"=w15) -> ("error out"=w34:errorcluster)  [unwired: 4 in, 4 out]
  n127 = call <userlib>:"DisposeApi.vi"("Error in"=w34) -> ()  [unwired: 10 in, 1 out]
  n128 = global write "GlobalesPrensa.vi" "Salir"(FALSE ("Salir")) -> ()
  n129 = while {
    tunnel: w66 -> [w376]
    tunnel: w65 -> [w375]
    tunnel: [w374] -> w64
    tunnel: [w373] -> w62
    tunnel: [w372] -> w90
    tunnel: [w371] -> w89
    tunnel: w88 -> [w370]
    tunnel: w87 -> [w369]
    shift-right: [w356] -> _
    shift-left: u32[] [] -> [w357]
    tunnel: w51 -> [w347]
    tunnel: [w355] -> w69
    tunnel: w6 -> [w353]
    shift-right: [w341] -> _
    shift-left: FALSE -> [_]
    stop <- w354 stop-if-true
    # "bar"
    # "volt"
    # "bar"
    # "volt"
    # "embolo"
    n130 = call <extravilib>:"Read.vi"("channel"=w347) -> ("element"=w283:T5)  [unwired: 1 in, 1 out]
    n131 = call <extravilib>:"Read.vi"("channel"=w353) -> ("element"=w354:bool)  [unwired: 1 in, 1 out]
    n132 = Tick Count (ms)() -> (millisecond timer value=w359:u32)
    n133 = feedback #4(w359) -> (w360:u32)
    n134 = feedback-in #4(w359) -> ()
    n135 = call-poly <vilib>:"DAQmx Read.vi"("task/channels in"=w376, "number of samples per channel"=4000, "error in"=w375) -> ("task out"=w374:refnum<k21>, "data"=w368:waveform(dbl)[], "error out"=w373:errorcluster)  [unwired: 10 in]
    n136 = Subtract(x=w359, y=w360) -> (x-y=w358:u32)
    "time/iteration (ms)" <- w358
    n137 = Split Signals(w368) -> (w364:dynamicdata, w367:dynamicdata, w366:dynamicdata, w365:dynamicdata)  [unwired: 4 in]
    n138 = call "Convert from Dynamic Data3"("Dynamic Data Type"=w366) -> ("Array"=w343:dbl[])  [unwired: 3 in]
    n139 = call "Convert from Dynamic Data4"("Dynamic Data Type"=w365) -> ("Array"=w342:dbl[])  [unwired: 3 in]
    n140 = call "Convert from Dynamic Data"("Dynamic Data Type"=w364) -> ("Array"=w345:dbl[])  [unwired: 3 in]
    n141 = call "Convert from Dynamic Data2"("Dynamic Data Type"=w367) -> ("Array"=w344:dbl[])  [unwired: 3 in]
    n142 = Build Array (concatenate)(w357, w358) -> (w356:u32[])
    n143 = call-poly <vilib>:"Mean.vi"("X"=w343) -> ("mean"=w289:dbl)  [unwired: 1 out]
    n144 = call-poly <vilib>:"Mean.vi"("X"=w342) -> ("mean"=w288:dbl)  [unwired: 1 out]
    n145 = call-poly <vilib>:"Mean.vi"("X"=w345) -> ("mean"=w287:dbl)  [unwired: 1 out]
    n146 = call-poly <vilib>:"Mean.vi"("X"=w344) -> ("mean"=w285:dbl)  [unwired: 1 out]
    n147 = expression code="15*x"(w287) -> (w286:dbl)
    n148 = expression code="20*x"(w285) -> (w284:dbl)
    n149 = Unbundle By Name(w283) -> ("Rampa (mm/min)"=w352:dbl, "Rampa (kN/min)"=w351:dbl, "Limite posicion (mm)"=w322:dbl, "Limite fuerza (kN)"=w350:dbl, "Posicion deseada (mm)"=w349:dbl, "Fuerza deseada (kN)"=w348:dbl, "Tiempo carga (s)"=w329:dbl, "Iniciar ensayo"=w341:bool, "Tipo control"=w323:u16)
    n150 = case shown="1" w323 {
      tunnel: w352 -> [w388 _]
      tunnel: w349 -> [w387 _]
      tunnel: w348 -> [_ w390]
      tunnel: w351 -> [_ w391]
      tunnel: [w388 w391] -> w331
      tunnel: [w387 w390] -> w327
      tunnel: [w386 w389] -> w332
      tunnel: w322 -> [w386 _]
      tunnel: w350 -> [_ w389]
      frame 0, Default {
      }
      frame 1 {
      }
    }
    n151 = Select(t=10.0, s=w341, f=0.0) -> (s? t:f=w333:dbl)
    n152 = call "TIME.vi"("Numeric 2"=0, "y"=w333) -> ("Numeric"=w328:dbl)
    n153 = expression code="(x-1.9826)*12.5"(w289) -> (w282:dbl)
    n154 = expression code="(x-1.9682)*50"(w288) -> (w281:dbl)
    n155 = formula code="/* PARAMETROS AVANZADOS DEL CONTROLADOR\n   Solo se usan los valores del panel si 'cod' (codigo de acceso) = 2026;\n   si no, se usan los valores por defecto. Se limitan a rangos seguros. */\nfloat64 P[8];\nif (cod==2026) {\n  P[0]=max(1,min(100,Kx));       /* ganancia lazo de posicion (V/mm) */\n  P[1]=max(0.1,min(60,Tix));     /* tiempo integral (s) */\n  P[2]=max(0.05,min(5,Kf));      /* ancho de banda lazo de fuerza (1/s) */\n  P[3]=max(0.02,min(50,k0));     /* rigidez inicial (kN/mm) */\n  P[4]=max(0.05,min(0.9,caida)); /* caida de carga para falla (fraccion) */\n  P[5]=max(1,min(2,sobre));      /* sobrecarga para falla (x limite) */\n  act=1;\n} else {\n  P[0]=30; P[1]=1.5; P[2]=0.5; P[3]=1; P[4]=0.3; P[5]=1.2;\n  act=0;\n}\nP[5]=1.2; /*sobrecarga para falla\nP[6]=50;   /* velocidad de retorno (mm/min), todos los casos y modos de control */\nP[7]=40;   /* maxima variacion de salida (V/s) */"("cod"="Codigo acceso", "Kx"="Kx lazo posicion (V/mm)", "Tix"="Ti lazo posicion (s)", "Kf"="Kf lazo fuerza (1/s)", "k0"="Rigidez inicial (kN/mm)", "caida"="Caida para falla (0-1)", "sobre"="Sobrecarga falla (x limite)") -> ("P"=w318:dbl[], "act"=→"Parametros avanzados":dbl)
    n156 = Boolean To (0,1)(Boolean="Confirmar parametros") -> (0, 1=w303:i16)
    n157 = Boolean To (0,1)(Boolean="PARO DE EMERGENCIA") -> (0, 1=w304:i16)
    n158 = Boolean To (0,1)(Boolean="Sin proteccion de carga") -> (0, 1=w290:i16)
    n159 = feedback #5() -> (w324:dbl[])  [unwired: 1 in]
    n160 = call <vilib>:"High Resolution Relative Seconds.vi"() -> ("relative seconds"=w296:dbl)
    n161 = feedback #6() -> (w330:dbl)  [unwired: 1 in]
    n162 = feedback #7() -> (w334:dbl)  [unwired: 1 in]
    n163 = feedback #8() -> (w338:dbl)  [unwired: 1 in]
    n164 = feedback #9() -> (w336:dbl)  [unwired: 1 in]
    n165 = formula code="/* ===========================================================================\n   CONTROLADOR PRENSA FLUIDTEK v16 - cascada fuerza -> posicion\n   Formula Node de FluidtekPrensaCONidentLEDI_v15.vi  (un paso del lazo, ~20 ms)\n   ===========================================================================\n\n   QUE HACE\n     1. Genera la consigna sp segun el estado st (maquina de estados).\n     2. Lazo externo: convierte sp (posicion o fuerza) en consigna de posicion\n        x_ref. En fuerza se divide por la rigidez estimada rig [kN/mm].\n     3. Lazo interno: PI de posicion -> comando u [V] a la servovalvula.\n     4. Protecciones: celda (F_corte), sobrecarga, caida de carga, limite de\n        posicion, paro de emergencia, presiones (desactivado) y NaN.\n\n   ESTADOS  st      0 reposo/aproximacion   1 carga   2 mantener   3 descarga\n                    4 retorno/fin           5 FALLA\n   CAUSAS   causa   0 ninguna  1 caida de carga  2 sobrecarga  3 limite de posicion\n                    4 paro de emergencia  5 limite de la celda (F_corte)\n                    7 limite por presiones (pa >= pa_max o F_pres >= F_corte)\n   MODOS    modo    0 control de desplazamiento [mm]    1 control de fuerza [kN]\n\n   TERMINALES (el nombre es el del terminal en la VI)\n     Entradas  x        posicion del vastago [mm]\n               F        fuerza de la celda [kN]\n               modo     ver arriba\n               t, tr    tiempo del ensayo [s] y reloj de alta resolucion [s]\n               pa       presion camara A, SIN vastago [bar]  (TR44.2, ai2)\n               pb       presion camara B, CON vastago [bar]  (TR49.2, ai3)\n                        (llegan en bar reales; el escalado esta en el diagrama:\n                         pa = (V_ai2 - 1.9826)*12.5   pb = (V_ai3 - 1.9682)*50)\n               vjog     velocidad de aproximacion fuera de ensayo [mm/min]\n               Flib     limite de fuerza fuera de ensayo [kN]\n               sinprot  1 = sin proteccion de carga fuera de ensayo\n               ini      INICIAR (>= 5 activo)      inip   valor anterior de ini\n               conf     'Confirmar parametros'\n               spm      consigna manual fuera de ensayo [mm o kN]\n               lim      consigna final del ensayo  rate   rampa [unidad/min]\n               tc       tiempo de mantenimiento [s]   xlim limite de posicion [mm]\n               paro     paro de emergencia\n               stp, f0p, tsp   st, f0 y ts del paso anterior\n               P        parametros avanzados (arreglo, >= 8)\n               S        estado persistente (arreglo de 12)\n               tkq, tqx SIN USO (vigilancia del QuantumX, retirada en v16)\n     Salidas   st, f0, ts, inio, sp, prot, prog, trest, falla, causa,\n               Fpko, xspo, kho, u, So (estado, 12), Lg (registro, 15)\n\n   PARAMETROS P[]  (si P trae menos de 8 elementos se usan los de entre parentesis)\n     P[0] Kx  ganancia del PI de posicion [V/mm] (30)    P[1] Tix tiempo integral [s] (1.5)\n     P[2] Kf  correccion del lazo de fuerza [1/s] (0.5)  P[3] rigidez inicial [kN/mm] (1)\n     P[4] caida de carga que dispara FALLA 1, fraccion del pico (0.3)\n     P[5] sobrecarga que dispara FALLA 2, fraccion de lim (1.2)\n     P[6] velocidad de retorno [mm/min] (50)             P[7] variacion maxima de u [V/s] (40)\n\n   ESTADO PERSISTENTE S[] -> So[]  (llega como 12 ceros en la primera iteracion)\n     0 x_ref  1 rig   2 F_pico   3 integ   4 sp_prev   5 t_prev\n     6 F_ref  7 x_ref_rig  8 x_inicio  9 u_prev  10 modo_prev  11 causa_act\n\n   REGISTRO Lg[]\n     0 t  1 st  2 sp  3 F  4 x  5 x_ref  6 u  7 rig  8 dt  9 falla  10 causa\n     11 prot  12 pa  13 pb  14 F_pres\n\n   PARO: salida 0 V, controlador en seguimiento (sin salto al soltarlo).\n   El historial de versiones esta en git (git log -- labview_control_software/PID.c).\n   v16: misma logica que v15, verificada paso a paso con 320 000+ pasos\n        aleatorios; solo cambian nombres, orden de la cabecera y se retira el\n        codigo muerto del QuantumX (causa 6).\n   =========================================================================== */\n\n\n/* ---------------------------------------------------------------------------\n   0. DECLARACIONES Y CONSTANTES\n   (el Formula Node no tiene #define: las constantes son variables)\n   --------------------------------------------------------------------------- */\n\n/* parametros de P */\nfloat64 Kx, Tix, Kf, rig_ini, frac_caida, frac_sobre, v_retorno, du_max;\n/* estado persistente (S) */\nfloat64 x_ref, rig, F_pico, integ, sp_prev, t_prev, F_ref, x_ref_rig, x_inicio;\nfloat64 u_prev, modo_prev, causa_act;\n/* variables de trabajo */\nfloat64 med, ini_ef, dt, v_aprox, F_lib;\nfloat64 dif, vel_sp, paso_sp, dF_min, rig_nueva;\nfloat64 x_ref_ini, x_ref_prev, err, u_pi;\nfloat64 F_pres, lim_pres;\n/* arreglos de salida */\nfloat64 So[12];\nfloat64 Lg[15];\n/* constantes de seguridad y de ajuste */\nfloat64 F_corte, pa_max, prot_pres_on, v_des, u_max, x_win, v_lenta;\nfloat64 rig_min, rig_max, alfa_rig, frac_freno, frac_pico_min, margen_xlim;\nfloat64 dF_base, dx_min_rig, dx_sin_contacto;\nfloat64 cFpA, cFpB;\n/* codigos de estado y de causa */\nfloat64 ST_REPOSO, ST_CARGA, ST_MANTIENE, ST_DESCARGA, ST_RETORNO, ST_FALLA;\nfloat64 CAU_NINGUNA, CAU_CAIDA, CAU_SOBRECARGA, CAU_LIM_POS, CAU_PARO, CAU_FCORTE, CAU_PRESION;\n\nF_corte  = 160;     /* kN: corte por la celda. 160 kN ~ 80 bar con el cilindro 160/80: BAJAR (CLAUDE.md 6) */\npa_max   = 95;      /* bar: corte por presion de la camara A (el TR44.2 satura a 100 bar) */\nprot_pres_on = 0;   /* 0 = corte por presiones DESACTIVADO (desde 2026-11-03); 1 = activo */\nv_des    = 15;      /* kN/min: carga/descarga en fuerza fuera de ensayo y descarga en ensayo */\nu_max    = 10;      /* V: saturacion del comando (tambien umbral del anti-windup) */\nx_win    = 2;       /* mm: x_ref no se separa de x mas que esto */\nv_lenta  = 2;       /* mm/min: avance lento fuera de ensayo con compresion */\nrig_min  = 0.02;    /* kN/mm: rigidez estimada minima */\nrig_max  = 50;      /* kN/mm: rigidez estimada maxima */\nalfa_rig = 0.3;     /* filtro de la rigidez estimada */\nfrac_freno    = 0.25;   /* avance lento si F > frac_freno*F_lib (fuera de ensayo) */\nfrac_pico_min = 0.2;    /* la caida de carga solo cuenta si el pico fue > 20 % de lim */\nmargen_xlim   = 0.5;    /* mm: tolerancia sobre el limite de posicion xlim */\ndF_base         = 0.05; /* kN: cambio minimo de fuerza para actualizar la rigidez */\ndx_min_rig      = 0.002;/* mm: cambio minimo de posicion para actualizar la rigidez */\ndx_sin_contacto = 5;    /* mm: mas que esto sin cambio de F = sin contacto */\n\n/* Fp = A_A*pa - A_B*pb con el cilindro 160/80 mm (kN/bar = A[m2]*100):\n   A_A = 201.06 cm2 (camara A, sin vastago), A_B = 150.80 cm2 (camara B, con vastago) */\ncFpA = 2.0106;\ncFpB = 1.5080;\n\nST_REPOSO = 0;  ST_CARGA = 1;  ST_MANTIENE = 2;  ST_DESCARGA = 3;  ST_RETORNO = 4;  ST_FALLA = 5;\nCAU_NINGUNA = 0;  CAU_CAIDA = 1;  CAU_SOBRECARGA = 2;  CAU_LIM_POS = 3;\nCAU_PARO = 4;  CAU_FCORTE = 5;  CAU_PRESION = 7;\n\nif (sizeOfDim(P,0)>=8) {\n    Kx=P[0]; Tix=P[1]; Kf=P[2]; rig_ini=P[3];\n    frac_caida=P[4]; frac_sobre=P[5]; v_retorno=P[6]; du_max=P[7];\n} else {\n    Kx=30; Tix=1.5; Kf=0.5; rig_ini=1;\n    frac_caida=0.3; frac_sobre=1.2; v_retorno=50; du_max=40;\n}\n\n\n/* ---------------------------------------------------------------------------\n   1. MEDICION ACTUAL Y ESTADO PERSISTENTE\n   --------------------------------------------------------------------------- */\n\n/* medicion del modo activo: posicion [mm] o fuerza [kN] */\nmed = x;\nif (modo>0.5) med = F;\n\n/* el estado llega como 12 ceros en la primera iteracion: rig>0 indica estado valido */\nif (sizeOfDim(S,0)>=12 && S[1]>0) {\n    x_ref=S[0]; rig=S[1]; F_pico=S[2]; integ=S[3]; sp_prev=S[4]; t_prev=S[5];\n    F_ref=S[6]; x_ref_rig=S[7]; x_inicio=S[8]; u_prev=S[9]; modo_prev=S[10]; causa_act=S[11];\n} else {\n    x_ref=x; rig=rig_ini; F_pico=0; integ=0; sp_prev=med; t_prev=tr;\n    F_ref=F; x_ref_rig=x; x_inicio=x; u_prev=0; modo_prev=modo; causa_act=0;\n}\n\ndt = tr - t_prev;\nif (dt<=0 || dt>1) dt = 0.02;   /* lectura de tiempo invalida: usa el periodo nominal */\n\nx_ref_ini = x_ref;   /* x_ref al empezar el paso (la proteccion de fuerza lo restituye) */\nprot = 0;\nst = stp;  f0 = f0p;  ts = tsp;\n\n\n/* ---------------------------------------------------------------------------\n   2. MAGNITUDES DERIVADAS Y LIMITES\n   --------------------------------------------------------------------------- */\n\n/* fuerza estimada por las presiones [kN] y corte por presiones (hoy desactivado) */\nF_pres = cFpA*pa - cFpB*pb;\nlim_pres = 0;\nif (prot_pres_on>0.5 && (pa>=pa_max || F_pres>=F_corte)) lim_pres = 1;\n\n/* velocidad de aproximacion [mm/min] y limite de fuerza fuera de ensayo [kN] */\nv_aprox = vjog;\nif (v_aprox<=0) v_aprox = 25;\nv_aprox = min(50,v_aprox);\n\nF_lib = abs(Flib);\nif (F_lib<=0) F_lib = 4;\nF_lib = max(0.2,min(50,F_lib));\n\n\n/* ---------------------------------------------------------------------------\n   3. INICIO DEL ENSAYO\n   INICIAR solo arranca el ensayo si 'Confirmar parametros' esta activo al\n   pulsarlo; si se rechaza, queda bloqueado (-1) hasta soltar INICIAR.\n   --------------------------------------------------------------------------- */\nini_ef = ini;\nif (ini>=5 && inip<5 && conf<0.5) ini_ef = -1;\nif (ini>=5 && inip<0) ini_ef = -1;\ninio = ini_ef;\n\n/* reinicio sin salto al iniciar o al cambiar el tipo de control */\nif ((ini_ef>=5 && inip<5) || modo!=modo_prev) {\n    x_ref = x;\n    integ = 0;\n    sp_prev = med;\n}\n\n\n/* ---------------------------------------------------------------------------\n   4. GENERADOR DE CONSIGNA sp (maquina de estados)\n   --------------------------------------------------------------------------- */\nif (ini_ef<5) {\n    /* FUERA DE ENSAYO: avance a v_aprox, retorno a v_retorno. Lento solo si se\n       avanza con compresion (F > frac_freno*F_lib); el retorno nunca se frena.\n       En fuerza, la consigna spm se limita a +-F_lib (o +-F_corte si sinprot). */\n    st = ST_REPOSO;\n    causa_act = CAU_NINGUNA;\n    if (modo>0.5) {\n        if (sinprot>0.5) {\n            dif = max(-F_corte,min(F_corte,spm)) - sp_prev;\n        } else {\n            dif = max(-F_lib,min(F_lib,spm)) - sp_prev;\n        }\n        vel_sp = v_des;\n        paso_sp = vel_sp*dt/60;\n        if (paso_sp<=0) paso_sp = 1e9;\n    } else {\n        dif = spm - sp_prev;\n        vel_sp = v_aprox;\n        if (dif<0) vel_sp = v_retorno;\n        if (sinprot<0.5 && dif>0 && F>frac_freno*F_lib) vel_sp = min(v_aprox,v_lenta);\n        paso_sp = vel_sp*dt/60;\n    }\n    /* la consigna sigue a spm con pendiente limitada a paso_sp por paso */\n    sp = sp_prev + max(-paso_sp,min(paso_sp,dif));\n} else {\n    /* EN ENSAYO */\n    if (inip<5) {\n        /* primer paso del ensayo: arranca la carga desde la medicion actual */\n        st = ST_CARGA;\n        f0 = med;\n        ts = t;\n        F_pico = 0;\n        F_ref = F;\n        x_ref_rig = x;\n        x_inicio = x;\n        causa_act = CAU_NINGUNA;\n    }\n    dif = lim - f0;\n    if (st==ST_CARGA) {\n        /* carga: rampa hacia lim */\n        sp = f0 + sign(dif)*abs(rate)*(t-ts)/60;\n        if (dif*(sp-lim)>=0) { sp=lim; st=ST_MANTIENE; ts=t; }\n    } else if (st==ST_MANTIENE) {\n        /* mantener lim durante tc segundos */\n        sp = lim;\n        if (t-ts>=tc) { st=ST_DESCARGA; ts=t; }\n    } else if (st==ST_DESCARGA) {\n        /* descarga: a v_retorno [mm/min] en desplazamiento, a v_des [kN/min] en fuerza */\n        vel_sp = v_des;\n        if (modo<0.5) vel_sp = v_retorno;\n        sp = lim - sign(dif)*vel_sp*(t-ts)/60;\n        if (dif*(f0-sp)>=0) { sp=f0; st=ST_RETORNO; ts=t; }\n    } else {\n        /* retorno/fin (4) o FALLA (5): consigna en el valor inicial */\n        sp = f0;\n    }\n}\n\n\n/* ---------------------------------------------------------------------------\n   5. RIGIDEZ ESTIMADA rig = dF/dx\n   En linea en todo momento salvo retorno y falla (reposo, aproximacion, carga,\n   mantenimiento y descarga, en ambos modos): asi el lazo de fuerza usa la\n   rigidez real.\n   --------------------------------------------------------------------------- */\ndF_min = dF_base;\nif (ini_ef>=5) dF_min = max(dF_base,dF_base*abs(lim-f0));\nif (st<=ST_DESCARGA && abs(F-F_ref)>dF_min && abs(x-x_ref_rig)>dx_min_rig) {\n    rig_nueva = (F-F_ref)/(x-x_ref_rig);\n    if (rig_nueva>rig_min) rig = rig + alfa_rig*(rig_nueva-rig);\n    F_ref = F;\n    x_ref_rig = x;\n}\nif (abs(x-x_ref_rig)>dx_sin_contacto) { F_ref=F; x_ref_rig=x; }   /* sin contacto: reinicia la referencia */\nrig = max(rig_min,min(rig_max,rig));\n\n\n/* ---------------------------------------------------------------------------\n   6. LAZO EXTERNO: consigna de posicion x_ref\n   --------------------------------------------------------------------------- */\nif (modo>0.5) {\n    /* control de fuerza */\n    if (st==ST_RETORNO) {\n        /* retorno a la posicion inicial x_inicio a v_retorno */\n        x_ref = x_ref + sign(x_inicio-x_ref)*min(abs(x_inicio-x_ref),v_retorno*dt/60);\n    } else if (st!=ST_FALLA) {\n        /* prealimentacion de la rampa + correccion normalizada por rigidez */\n        x_ref_prev = x_ref;\n        x_ref = x_ref + (sp-sp_prev)/rig + Kf*(sp-F)/rig*dt;\n        /* velocidad maxima del piston = v_aprox (evita embalarse sin contacto) */\n        if (st<=ST_DESCARGA) x_ref = x_ref_prev + max(-v_aprox*dt/60,min(v_aprox*dt/60,x_ref-x_ref_prev));\n    }\n} else {\n    /* control de desplazamiento */\n    if (st!=ST_FALLA) x_ref = sp;\n}\n\n\n/* ---------------------------------------------------------------------------\n   7. PROTECCION DE FUERZA FUERA DE ENSAYO\n   Con compresion F > F_lib no deja avanzar; retroceder (alejarse) siempre esta\n   permitido.\n   --------------------------------------------------------------------------- */\nif (st==ST_REPOSO && sinprot<0.5) {\n    if (F>F_lib) { x_ref=min(x_ref,x_ref_ini); integ=min(integ,0); prot=1; }\n    if (prot>0.5 && modo<0.5) sp = x_ref;\n}\n\n\n/* ---------------------------------------------------------------------------\n   8. DETECCION DE FALLA, LIMITES Y PARO DE EMERGENCIA\n   --------------------------------------------------------------------------- */\nif (st>=ST_CARGA && st<=ST_DESCARGA) {\n    F_pico = max(F_pico,F);\n    if (modo>0.5 && st<=ST_MANTIENE && F_pico>frac_pico_min*abs(lim) && F<(1-frac_caida)*F_pico) {\n        st=ST_FALLA; causa_act=CAU_CAIDA; x_ref=x;           /* caida de carga */\n    } else if (modo>0.5 && F>frac_sobre*abs(lim)) {\n        st=ST_FALLA; causa_act=CAU_SOBRECARGA; x_ref=x;      /* sobrecarga */\n    } else if (x>xlim+margen_xlim) {\n        st=ST_FALLA; causa_act=CAU_LIM_POS; x_ref=x;         /* limite de posicion */\n    }\n}\n/* limite del sistema: en ensayo se declara FALLA */\nif (st>=ST_CARGA && st<=ST_RETORNO && abs(F)>=F_corte) { st=ST_FALLA; causa_act=CAU_FCORTE;  x_ref=x; }\nif (st>=ST_CARGA && st<=ST_RETORNO && lim_pres>0.5)    { st=ST_FALLA; causa_act=CAU_PRESION; x_ref=x; }\nif (paro>0.5 && ini_ef>=5)                             { st=ST_FALLA; causa_act=CAU_PARO; }\nif (st==ST_FALLA) sp = med;\nif (modo>0.5) sp = max(-F_corte,min(F_corte,sp));   /* consigna de fuerza nunca sobre el corte */\n\n\n/* ---------------------------------------------------------------------------\n   9. LAZO INTERNO DE POSICION (PI con anti-windup) Y SEGURIDADES DE SALIDA\n   --------------------------------------------------------------------------- */\nx_ref = max(x-x_win,min(x+x_win,x_ref));\nerr = x_ref - x;\nu_pi = Kx*(err+integ/Tix);\nif (abs(u_pi)<u_max) integ = integ + err*dt;                 /* integra solo si no satura */\nu = max(-u_max,min(u_max,u_pi));\nu = max(u_prev-du_max*dt,min(u_prev+du_max*dt,u));           /* limite de variacion (V/s) */\n\n/* LIMITE DEL SISTEMA: desde F_corte no se permite empujar mas, en cualquier estado y modo */\nif (F>=F_corte)  { u=min(u,0); integ=min(integ,0); x_ref=min(x_ref,x); prot=1; }\nif (F<=-F_corte) { u=max(u,0); integ=max(integ,0); x_ref=max(x_ref,x); prot=1; }\n/* corte por presiones (solo si prot_pres_on = 1) */\nif (lim_pres>0.5) { u=min(u,0); integ=min(integ,0); x_ref=min(x_ref,x); prot=1; }\n/* PARO: 0 V y seguimiento, para que al soltarlo no haya salto */\nif (paro>0.5) { u=0; integ=0; x_ref=x; sp=med; }\n\n\n/* ---------------------------------------------------------------------------\n   10. INDICADORES PARA LA INTERFAZ\n   --------------------------------------------------------------------------- */\nprog = 0;\ntrest = 0;\nif (st==ST_MANTIENE) {\n    if (tc>0) prog = 100*min(1,(t-ts)/tc);\n    trest = max(0,tc-(t-ts));\n}\nif (st==ST_DESCARGA || st==ST_RETORNO) prog = 100;\nfalla = 0;\nif (st==ST_FALLA) falla = 1;\ncausa = causa_act;\nif (paro>0.5) { causa=CAU_PARO; falla=1; }   /* alarma de PARO tambien fuera de ensayo */\nFpko = F_pico;\n\n\n/* ---------------------------------------------------------------------------\n   11. ESTADO PARA EL SIGUIENTE PASO Y REGISTRO\n   --------------------------------------------------------------------------- */\nsp_prev = sp;\nu_prev = u;\nt_prev = tr;\nmodo_prev = modo;\n\nSo[0]=x_ref;  So[1]=rig;       So[2]=F_pico;  So[3]=integ;     So[4]=sp_prev; So[5]=t_prev;\nSo[6]=F_ref;  So[7]=x_ref_rig; So[8]=x_inicio; So[9]=u_prev;   So[10]=modo_prev; So[11]=causa_act;\nxspo = x_ref;\nkho = rig;\n\nLg[0]=t;    Lg[1]=st;   Lg[2]=sp;   Lg[3]=F;   Lg[4]=x;   Lg[5]=x_ref;\nLg[6]=u;    Lg[7]=rig;  Lg[8]=dt;   Lg[9]=falla; Lg[10]=causa; Lg[11]=prot;\nLg[12]=pa;  Lg[13]=pb;  Lg[14]=F_pres;\n\n\n/* ---------------------------------------------------------------------------\n   12. PROTECCION ANTE NaN\n   Lectura invalida del cDAQ (NaN en posicion o fuerza): salida 0 V, FALLA en\n   ensayo y reinicio del estado (So[1]=0 hace que el proximo paso lo descarte).\n   --------------------------------------------------------------------------- */\nif (!(x==x) || !(F==F)) {\n    u = 0;\n    falla = 1;\n    So[1] = 0;\n    if (st>=ST_CARGA && st<=ST_RETORNO) st = ST_FALLA;\n    Lg[6] = 0;\n    Lg[9] = 1;\n}"("ini"=w333, "lim"=w332, "rate"=w331, "tc"=w329, "t"=w328, "spm"=w327, "stp"=w330, "f0p"=w338, "tsp"=w336, "inip"=w334, "F"=w284, "x"=w286, "modo"=w323, "xlim"=w322, "S"=w324, "P"=w318, "paro"=w304, "conf"=w303, "tr"=w296, "vjog"="Vel. aproximacion (mm/min)", "Flib"="Fmax fuera de ensayo (kN)", "sinprot"=w290, "pa"=w282, "pb"=w281) -> ("sp"=w326:dbl, "st"=w295:dbl, "f0"=w339:dbl, "ts"=w337:dbl, "inio"=w335:dbl, "u"=w321:dbl, "So"=w325:dbl[], "xspo"=→"Consigna posicion interna (mm)":dbl, "kho"=→"Rigidez estimada (kN/mm)":dbl, "prog"=→"Progreso mantenimiento":dbl, "trest"=→"Tiempo restante carga (s)":dbl, "causa"=w301:dbl, "Fpko"=→"Carga maxima (kN)":dbl, "prot"=w298:dbl, "Lg"=w293:dbl[])  [unwired: 1 out]
    "Estado del ensayo" <- w295
    "Causa de la falla" <- w301
    "Lg log" <- w293
    n166 = feedback-in #5(w325) -> ()
    n167 = Bundle("Numeric"=w328, "mean"=w286, "mean"=w284, "mean"=w282, "mean"=w281, "sp"=w326) -> (w340:T6)  [unwired: 1 in]
    n168 = feedback-in #6(w295) -> ()
    n169 = feedback-in #7(w335) -> ()
    n170 = feedback-in #8(w339) -> ()
    n171 = feedback-in #9(w337) -> ()
    n172 = call-poly <vilib>:"DAQmx Write.vi"("task/channels in"=w370, "data"=w321, "error in"=w369) -> ("task out"=w372:refnum<k21>, "error out"=w371:errorcluster)  [unwired: 10 in, 1 out]
    n173 = Greater Than 0?(x=w301) -> (x > 0?=→"Falla":bool)
    n174 = Greater Than 0?(x=w298) -> (x > 0?=→"Proteccion de fuerza activa":bool)
    n175 = Greater Than 0?(x=w295) -> (x > 0?=w292:bool)
    n176 = case shown="True" w292 {
      tunnel: w293 -> [_ w384]
      frame False {
      }
      frame True {
        n177 = global read "GlobalesPrensa.vi" "ArchivoControl"() -> (w383:path)
        n178 = call-poly <vilib>:"Write Delimited Spreadsheet.vi"("file path (dialog if empty)"=w383, "format (%.3f)"="%.5f", "2D data"=dbl[][] [], "1D data"=w384, "append to file? (new file:F)"=TRUE, "error in (no error)"=errorcluster {"status"=FALSE, "code"=0, "source"=""}, "transpose? (no:F)"=FALSE, "delimiter (\\t)"="\t" ("delimiter (\\t)")) -> ()  [unwired: 6 in, 2 out]
      }
    }
    n179 = global write "GlobalesPrensa.vi" "Ensayando"(w292) -> ()
    n180 = call <vilib>:"Boolean Crossing PtByPt.vi"("input"=w292) -> ("crossing"=w294:bool)  [unwired: 2 in]
    n181 = case shown="True" w294 {
      frame False {
      }
      frame True {
        n182 = property on="Tenacidad en vigas" class="Ring (strict)"() -> ("RingText.Text"=w385:string)  [unwired: 2 in, 2 out]
        n183 = global write "GlobalesPrensa.vi" "InfoEnsayo"(w385) -> ()
      }
    }
    n184 = call <extravilib>:"Write.vi"("element"=w340) -> ("channel"=w355:T7)  [unwired: 1 out]
  }
  n185 = call <vilib>:"DAQmx Stop Task.vi"("task/channels in"=w64, "error in"=w62) -> ("task out"=w63:refnum<k21>, "error out"=w61:errorcluster)  [unwired: 12 in]
  n186 = call <vilib>:"DAQmx Stop Task.vi"("task/channels in"=w90, "error in"=w89) -> ("task out"=w91:refnum<k21>, "error out"=w92:errorcluster)  [unwired: 12 in]
  n187 = while {
    tunnel: [w392] -> w51
    tunnel: w69 -> [w413]
    tunnel: w6 -> [w433]
    shift-right: [w408] -> _
    shift-left: dbl[] [] -> [w410]
    shift-right: [w407] -> _
    shift-left: dbl[] [] -> [w409]
    stop <- w432 stop-if-true
    # "Bloqueo: APLICAR NORMA solo actua en reposo (0) o falla (5)"
    n188 = call <extravilib>:"Read.vi"("channel"=w433) -> ("element"=w432:bool)  [unwired: 1 in, 1 out]
    n189 = call <extravilib>:"Read.vi"("channel"=w413) -> ("element"=w422:T9)  [unwired: 1 in, 1 out]
    n190 = Unbundle(w422) -> ("Numeric"=→"Tiempo (s)":dbl, w411:dbl, w412:dbl, →"Presión A (bar)":dbl, →"Presión B (bar)":dbl, "Limite fuerza (kN)"=w418:dbl)
    "Fuerza actual (KN)" <- w412
    "Posicion actual (mm)" <- w411
    "Vertical Progress Bar" <- w411
    n191 = Insert Into Array(array=w410, new element=w411) -> (w408:dbl[])  [unwired: 1 in]
    n192 = Insert Into Array(array=w409, new element=w412) -> (w407:dbl[])  [unwired: 1 in]
    n193 = case shown="1" "Tipo ensayos" {
      tunnel: [w445 w455] -> w402
      frame 0, Default {
        n194 = property on="Flexotracción en losas" class="Ring (strict)"("Visible"=TRUE) -> ()  [unwired: 2 in, 2 out]
        n195 = property on="Velocidad norma (mm/min)" class="DigNum (strict)"("Visible"=TRUE) -> ()  [unwired: 2 in, 2 out]
        n196 = property on="Tenacidad en vigas" class="Ring (strict)"("Visible"=FALSE) -> ()  [unwired: 2 in, 2 out]
        n197 = property on="Velocidad norma (mm/min)  2" class="Str"("Visible"=FALSE) -> ()  [unwired: 2 in, 2 out]
        n198 = case shown="2" "Flexotracción en losas" {
          tunnel: [1.5 4.0 1.0 1.0] -> w445
          frame 0, Default {
          }
          frame 3 {
          }
          frame 2 {
          }
          frame 1 {
          }
        }
        "Velocidad norma (mm/min)" <- w445
      }
      frame 1 {
        n199 = property on="Tenacidad en vigas" class="Ring (strict)"("Visible"=TRUE) -> ()  [unwired: 2 in, 2 out]
        n200 = property on="Velocidad norma (mm/min)" class="DigNum (strict)"("Visible"=FALSE) -> ()  [unwired: 2 in, 2 out]
        n201 = property on="Velocidad norma (mm/min)  2" class="Str"("Visible"=TRUE) -> ()  [unwired: 2 in, 2 out]
        n202 = property on="Flexotracción en losas" class="Ring (strict)"("Visible"=FALSE) -> ()  [unwired: 2 in, 2 out]
        n203 = case shown="0, Default" "Tenacidad en vigas" {
          tunnel: ["0.05 - 0.1" "0.06 - 0.12" "0.1" "0.5 ± 0.05" "0.25"] -> w456
          frame 0, Default {
          }
          frame 1 {
          }
          frame 3 {
          }
          frame 4 {
          }
          frame 2 {
          }
        }
        "Velocidad norma (mm/min)  2" <- w456
        n204 = Fract/Exp String To Number(string=w456) -> (number=w455:dbl)  [unwired: 3 in, 1 out]
      }
    }
    n205 = Bundle(w408, w407) -> (→"fuerza desplazamiento":cluster{dbl[], dbl[]})  [unwired: 1 in]
    n206 = Wait (ms)(milliseconds to wait=u32 100) -> ()  [unwired: 1 out]
    n207 = local read "Estado del ensayo"() -> (w401:dbl)
    n208 = case shown="0, Default" "Tipo control" {
      tunnel: [w440 w444] -> w417
      tunnel: w412 -> [w439 w444]
      tunnel: w411 -> [w440 w443]
      frame 0, Default {
        n209 = local write "Fuerza deseada (kN)"(w439) -> ()
        n210 = property on="Fuerza deseada (kN)" class="DigNum (strict)"("DisabledEnum"=T8."Disabled" ("Disabled")) -> ()  [unwired: 2 in, 2 out]
        n211 = property on="Posicion deseada (mm)" class="Slide (strict)"("DisabledEnum"=T8."Enabled" ("Disabled")) -> ()  [unwired: 2 in, 2 out]
      }
      frame 1 {
        n212 = local write "Posicion deseada (mm)"(w443) -> ()
        n213 = property on="Fuerza deseada (kN)" class="DigNum (strict)"("DisabledEnum"=T8."Enabled" ("Disabled")) -> ()  [unwired: 2 in, 2 out]
        n214 = property on="Posicion deseada (mm)" class="Slide (strict)"("DisabledEnum"=T8."Disabled" ("Disabled")) -> ()  [unwired: 2 in, 2 out]
      }
    }
    n215 = Equal To 0?(x="Tipo control") -> (x = 0?=w405:bool)
    n216 = Not Equal To 0?(x="Tipo control") -> (x != 0?=w404:bool)
    n217 = Select(t=T8."Disabled" ("Disabled"), s="Iniciar ensayo", f=T8."Enabled" ("Disabled")) -> (s? t:f=w414:T8)
    n218 = In Range and Coerce(upper limit=4.5, x=w401, lower limit=0.5) -> (In Range?=w398:bool)  [unwired: 1 out]
    n219 = property on="Limite fuerza (kN)" class="DigNum (strict)"("DisabledEnum"=w414) -> ()  [unwired: 2 in, 2 out]
    n220 = property on="Rampa (kN/min)" class="DigNum (strict)"("DisabledEnum"=w414) -> ()  [unwired: 2 in, 2 out]
    n221 = property on="Rampa (mm/min)" class="DigNum (strict)"("Visible"=w405) -> ()  [unwired: 2 in, 2 out]
    n222 = property on="Limite fuerza (kN)" class="DigNum (strict)"("Visible"=w404) -> ()  [unwired: 2 in, 2 out]
    n223 = property on="Rampa (kN/min)" class="DigNum (strict)"("Visible"=w404) -> ()  [unwired: 2 in, 2 out]
    n224 = property on="Fuerza deseada (kN)" class="DigNum (strict)"("DisabledEnum"=w414) -> ()  [unwired: 2 in, 2 out]
    n225 = property on="Posicion deseada (mm)" class="Slide (strict)"("DisabledEnum"=w414) -> ()  [unwired: 2 in, 2 out]
    n226 = property on="Tiempo carga (s)" class="DigNum (strict)"("DisabledEnum"=w414) -> ()  [unwired: 2 in, 2 out]
    n227 = property on="Limite posicion (mm)" class="DigNum (strict)"("DisabledEnum"=w414) -> ()  [unwired: 2 in, 2 out]
    n228 = Not(x=w398) -> (.not. x?=w397:bool)
    n229 = And(x="Aplicar velocidad de norma", y=w397) -> (x .and. y?=w395:bool)
    n230 = case shown="False" w395 {
      tunnel: w402 -> [_ w435]
      frame False {
      }
      frame True {
        n231 = local write "Rampa (mm/min)"(w435) -> ()
        n232 = local write "Tipo control"(enum16{"Desplazamiento", "Fuerza"}."Desplazamiento" ("Tipo control")) -> ()
      }
    }
    n233 = Bundle("Rampa (mm/min)"="Rampa (mm/min)", "Rampa (kN/min)"="Rampa (kN/min)", "Limite posicion (mm)"="Limite posicion (mm)", "Limite fuerza (kN)"="Limite fuerza (kN)", "Posicion deseada (mm)"="Posicion deseada (mm)", "Fuerza deseada (kN)"="Fuerza deseada (kN)", "Tiempo carga (s)"="Tiempo carga (s)", "Iniciar ensayo"="Iniciar ensayo", "Tipo control"="Tipo control") -> (w393:T5)  [unwired: 1 in]
    n234 = Merge Signals(w418, w417) -> (→"control signals":dynamicdata)
    n235 = call <extravilib>:"Write.vi"("element"=w393) -> ("channel"=w392:T10)  [unwired: 1 out]
  }
  n236 = call <vilib>:"DAQmx Clear Task.vi"("task in"=w63, "error in"=w61) -> ("error out"=w85:errorcluster)  [unwired: 13 in]
  n237 = call <vilib>:"DAQmx Clear Task.vi"("task in"=w91, "error in"=w92) -> ("error out"=w86:errorcluster)  [unwired: 13 in]
  n238 = call <vilib>:"Simple Error Handler.vi"("error in (no error)"=w85) -> ()  [unwired: 4 in, 5 out]
  n239 = call <vilib>:"Simple Error Handler.vi"("error in (no error)"=w86) -> ()  [unwired: 4 in, 5 out]
